vi "Get Memory Data.vi"(8 "error in (no error)":errorcluster caption="错误输入（无错误）", 11 "nDevId":i32) -> (0 "error out":errorcluster caption="错误输出", 3 "function return":u32)   [LabVIEW 2017, in "smncsftmt.lvlib"]
doc: "__declspec(dllexport) FtmtRawData* GetMemoryData(int nDevId);"
uses:
  smncsftmt.lvlib
  smncsftmt.dll
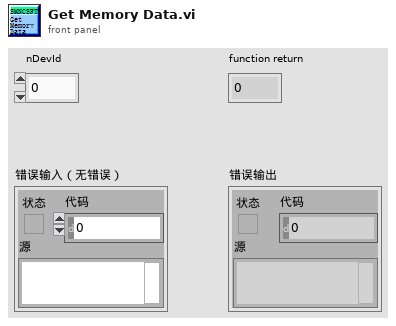
[diagram p1: front panel]
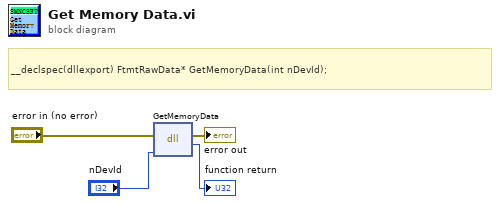
[diagram p0: block diagram]
diagram:
  # "__declspec(dllexport) FtmtRawData* GetMemoryData(int nDevId);"
  n1 = dll-call lib="PTH2oabs CUsersaDesktop\nLABVIEW范例National InstrumentsLabVIEW 2017user.lib\tsmncsftmtsmncsftmt.*" fn="GetMemoryData"(error in="error in (no error)", "nDevId"="nDevId") -> (error out=→"error out":errorcluster, →"function return":u32)  [unwired: 3 in, 1 out]
